vi "Read current vs temperature_3ch_2.1.vi"(8 "stop":bool) -> (0 "X3":cluster{"Y":dbl[], "Y":dbl[]}[](graph), 1 "Zx 4":cluster{"Y":dbl[], "Y":dbl[]}[](graph), 2 "Zx 3":cluster{"Y":dbl[], "Y":dbl[]}[](graph), 3 "Temp vs Time":cluster{"Y":dbl[], "Y":dbl[]}[](graph), 4 "i X":cluster{"Y":dbl[], "Y":dbl[]}[](graph), 5 "X 2":cluster{"Y":dbl[], "Y":dbl[]}[](graph))   [LabVIEW 2011]
uses:
  SubVI/ITX_Global.vi
  DAQ-lockin-SubVI/Source/Lock-in Globles.vi
panel:
  in  "Tab Control":T1(tab)
  in  "Lock-in # 2":u16(ring)=1 items=["Lock-in #1", "Lock-in #2", "Lock-in #3", "Lock-in #4"]
  out "OSC Configuration":T2(array[cluster])=[{"Signal Type"=enum."Sine Wave", "DC"=0.0005, "Amplitude"=0.001, "frequency"=1.346, "Phase"=0.0}, {"Signal Type"=enum."Sine Wave", "DC"=0.0, "Amplitude"=0.0, "frequency"=1.346, "Phase"=0.0}, {"Signal Type"=enum."Sine Wave", "DC"=0.0, "Amplitude"=0.0, "frequency"=1.346, "Phase"=0.0}, {"Signal Type"=enum."Sine Wave", "DC"=0.0, "Amplitude"=0.0, "frequency"=1.346, "Phase"=0.0}] {"frequency" format="%0.2p"; "Amplitude" format="%0.2p"; "DC" format="%.2p"}
  in  "Lock-in # 1":u16(ring) items=["Lock-in #1", "Lock-in #2", "Lock-in #3", "Lock-in #4"]
  in  "Lock-in # 3":u16(ring)=2 items=["Lock-in #1", "Lock-in #2", "Lock-in #3", "Lock-in #4"]
  in  "Lock-in # 4":u16(ring)=3 items=["Lock-in #1", "Lock-in #2", "Lock-in #3", "Lock-in #4"]
  in  "milliseconds to wait":u32=1000
  in  "Comments":string="SA02610M 20130128\ncool down\n"
  out "Connected":string="I-:4\nV2+:28\nI+:1\nV1+:2\nV-:3\nV2-:5\n"
  out "i Y":cluster{"Y":dbl[], "Y":dbl[]}[](graph)
  out "i X 3":cluster{"Y":dbl[], "Y":dbl[]}[](graph)
  out "i Y 3":cluster{"Y":dbl[], "Y":dbl[]}[](graph)
  out "Y 2":cluster{"Y":dbl[], "Y":dbl[]}[](graph)
  out "Y3":cluster{"Y":dbl[], "Y":dbl[]}[](graph)
  out "Zy 3":cluster{"Y":dbl[], "Y":dbl[]}[](graph)
  out "Zy 4":cluster{"Y":dbl[], "Y":dbl[]}[](graph)
  out "i X 2":cluster{"Y":dbl[], "Y":dbl[]}[](graph)
  out "i X 4":cluster{"Y":dbl[], "Y":dbl[]}[](graph)
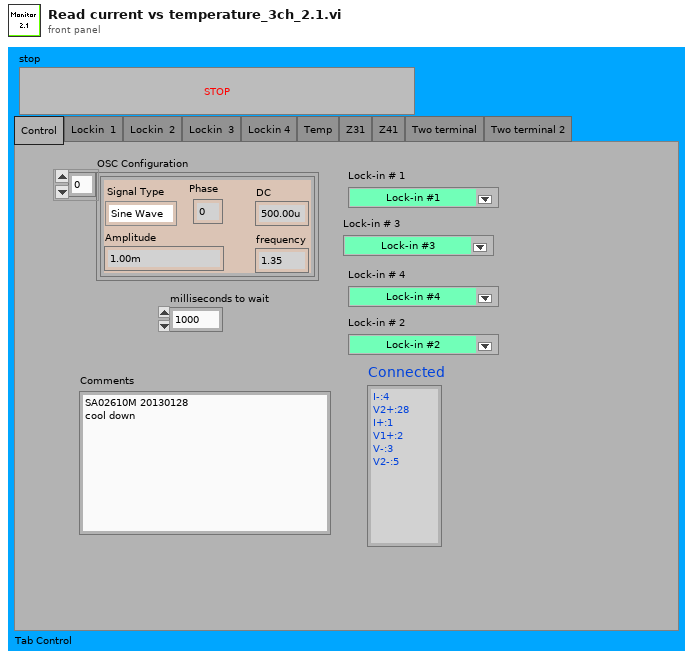
[diagram p1: front panel]
types:
  T1 = enum32{"Control", "Lockin  1", "Lockin  2", "Lockin  3", "Lockin 4", "Temp", "Z31", "Z41", "Two terminal", "Two terminal 2"}
  T2 = cluster{"Signal Type":enum16{"Sine Wave", "Triangle Wave", "Square Wave", "Sawtooth Wave"}, "DC":dbl, "Amplitude":dbl, "frequency":dbl, "Phase":dbl}[]
  T3 = cluster{"Signal Type":enum16{"Sine Wave", "Triangle Wave", "Square Wave", "Sawtooth Wave"}, "DC":dbl, "Amplitude":dbl, "frequency":dbl, "Phase":dbl}
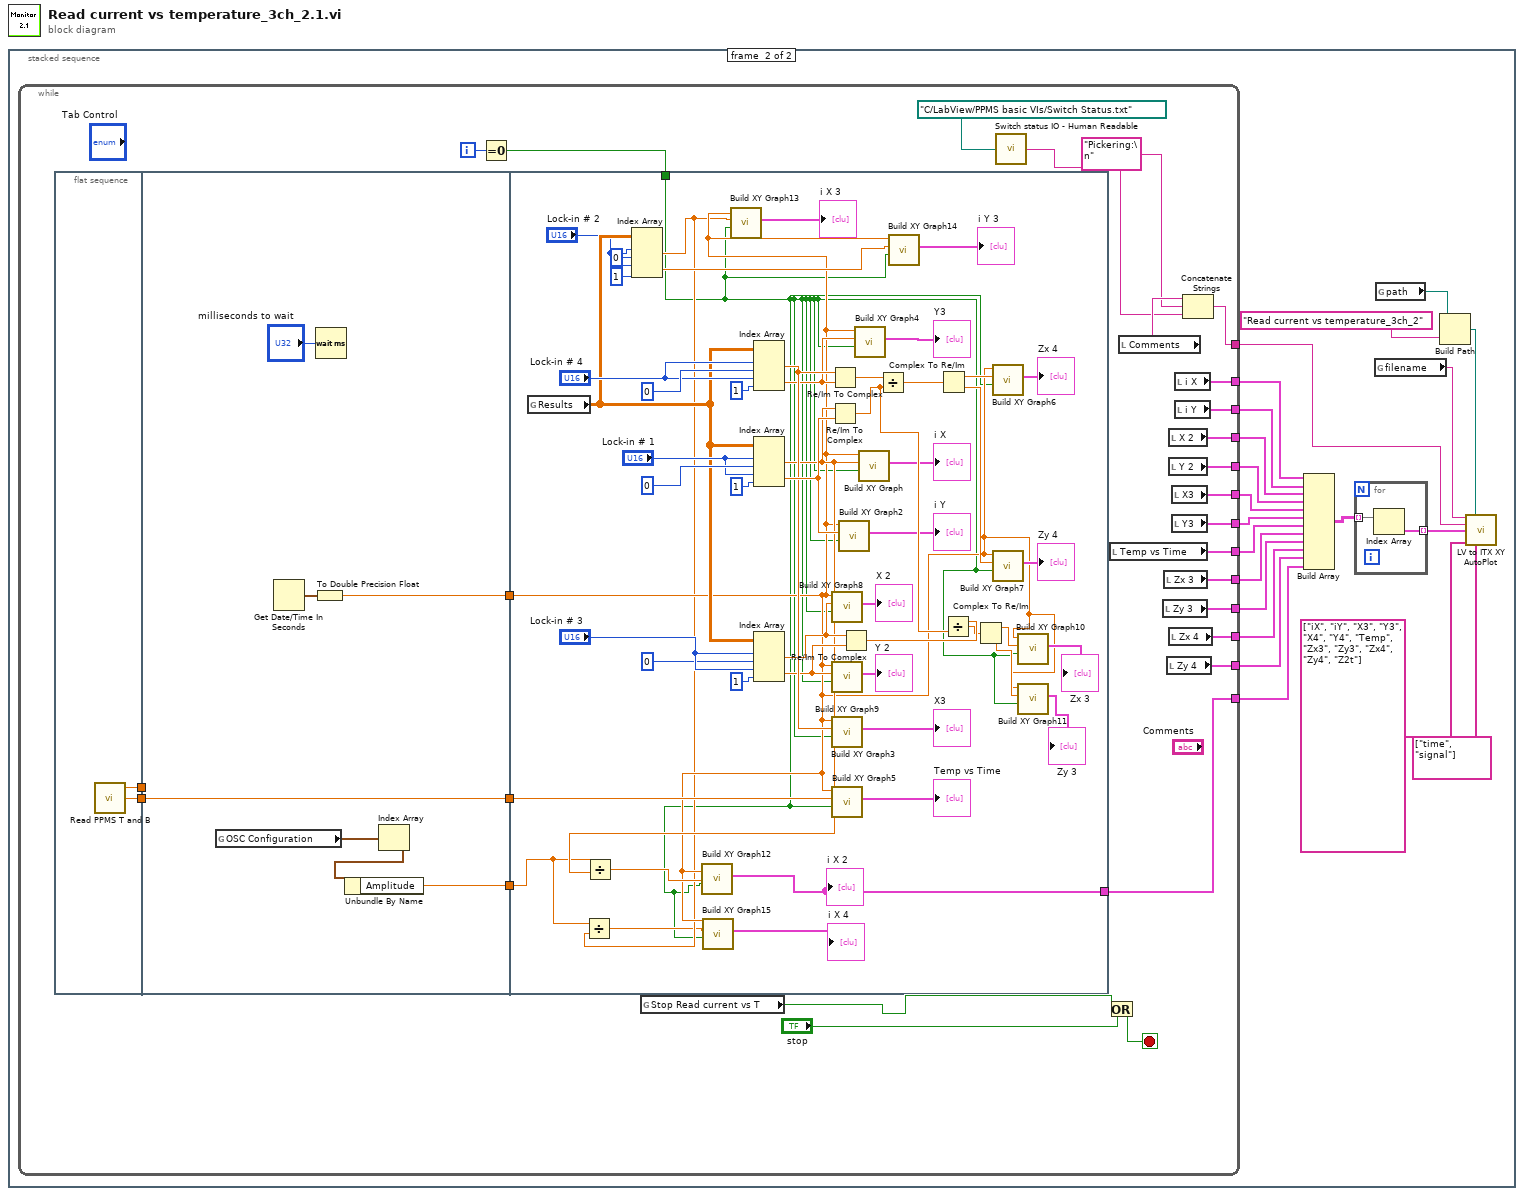
[diagram p0: block diagram]
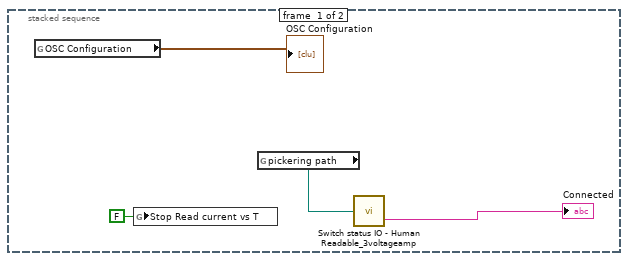
[diagram p2: hidden frame]
diagram:
  n1 = stacked-sequence {
    frame #0 {
      n2 = global read "Lock-in Globles.vi" "OSC Configuration"() -> (→"OSC Configuration":T2)
      n3 = global write "Lock-in Globles.vi" "Stop Read current vs T"(FALSE ("Stop Read current vs T")) -> ()
      n4 = global read "ITX_Global.vi" "pickering path"() -> (w1:path)
      n5 = call <userlib>:"Switch status IO - Human Readable_3voltageamp.vi"("Switch status"=w1) -> ("String"=→"Connected":string)  [unwired: 3 in]
    }
    frame #1 {
      n6 = while {
        tunnel: [w46] -> w25
        tunnel: [w45] -> w24
        tunnel: [w44] -> w23
        tunnel: [w43] -> w22
        tunnel: [w42] -> w21
        tunnel: [w41] -> w20
        tunnel: [w40] -> w19
        tunnel: [w39] -> w18
        tunnel: [w38] -> w17
        tunnel: [w37] -> w16
        tunnel: [w36] -> w15
        tunnel: [w34] -> w11
        tunnel: [w28] -> w5
        i -> [w52]
        stop <- w48 stop-if-true
        n7 = flat-sequence {
          tunnel: [w56] -> w53
          tunnel: [w55] -> w49
          tunnel: [w62] -> w54
          tunnel: w53 -> [w62]
          tunnel: [w60] -> w50
          tunnel: w49 -> [_]
          tunnel: [w57] -> w29
          tunnel: w54 -> [w96]
          tunnel: w51 -> [w65]
          tunnel: w50 -> [w69]
          tunnel: w29 -> [w68]
          tunnel: [w77] -> w28
          frame #0 {
            n8 = call "Read PPMS T and B.vi"() -> ("Temperature"=w56:dbl, "Time"=w55:dbl)  [unwired: 3 in, 1 out]
          }
          frame #1 {
            n9 = global read "Lock-in Globles.vi" "OSC Configuration"() -> (w59:T2)
            n10 = Get Date/Time In Seconds() -> (seconds since 1Jan1904=w61:timestamp)
            n11 = To Double Precision Float(number=w61) -> (double precision float=w60:dbl)
            n12 = Wait (ms)(milliseconds to wait="milliseconds to wait") -> ()  [unwired: 1 out]
            n13 = Index Array(array=w59) -> (element=w58:T3)  [unwired: 1 in]
            n14 = Unbundle By Name(w58) -> ("Amplitude"=w57:dbl)
          }
          frame #2 {
            n15 = global read "Lock-in Globles.vi" "Results"() -> (w76:dbl[][])
            n16 = Index Array(array=w76, index (row) #1="Lock-in # 2", index (col) #1=0 ("disabled index (col)"), index (row) #2="Lock-in # 2", index (col) #2=1 ("disabled index (col)")) -> (element #1=w67:dbl, element #2=w70:dbl)
            n17 = Divide(x=w68, y=w67) -> (x/y=w66:dbl)
            n18 = call "Build XY Graph15"("Reset"=w65, "Y Input"=w66, "X Input"=w69) -> ("XY Graph"=→"i X 4":cluster{"Y":dbl[], "Y":dbl[]}[])  [unwired: 2 in, 6 out]
            n19 = call "Build XY Graph13"("Reset"=w65, "Y Input"=w67, "X Input"=w69) -> ("XY Graph"=→"i X 3":cluster{"Y":dbl[], "Y":dbl[]}[])  [unwired: 2 in, 6 out]
            n20 = Index Array(array=w76, index (row) #1="Lock-in # 4", index (col) #1=0 ("disabled index (col)"), index (row) #2="Lock-in # 4", index (col) #2=1 ("disabled index (col)")) -> (element #1=w104:dbl, element #2=w103:dbl)
            n21 = Index Array(array=w76, index (row) #1="Lock-in # 1", index (col) #1=0 ("disabled index (col)"), index (row) #2="Lock-in # 1", index (col) #2=1 ("disabled index (col)")) -> (element #1=w79:dbl, element #2=w105:dbl)
            n22 = Divide(x=w68, y=w79) -> (x/y=w78:dbl)
            n23 = call "Build XY Graph12"("Reset"=w65, "Y Input"=w78, "X Input"=w69) -> ("XY Graph"=w77:cluster{"Y":dbl[], "Y":dbl[]}[])  [unwired: 2 in, 6 out]
            "i X 2" <- w77
            n24 = Index Array(array=w76, index (row) #1="Lock-in # 3", index (col) #1=0 ("disabled index (col)"), index (row) #2="Lock-in # 3", index (col) #2=1 ("disabled index (col)")) -> (element #1=w90:dbl, element #2=w89:dbl)
            n25 = Re/Im To Complex(1:w103, 2:w104) -> (0:w102:cdb)
            n26 = Re/Im To Complex(1:w105, 2:w79) -> (0:w87:cdb)
            n27 = call "Build XY Graph8"("Reset"=w65, "Y Input"=w90, "X Input"=w69) -> ("XY Graph"=→"X 2":cluster{"Y":dbl[], "Y":dbl[]}[])  [unwired: 2 in, 6 out]
            n28 = call "Build XY Graph9"("Reset"=w65, "Y Input"=w89, "X Input"=w69) -> ("XY Graph"=→"Y 2":cluster{"Y":dbl[], "Y":dbl[]}[])  [unwired: 2 in, 6 out]
            n29 = call "Build XY Graph3"("Reset"=w65, "Y Input"=w104, "X Input"=w69) -> ("XY Graph"=→"X3":cluster{"Y":dbl[], "Y":dbl[]}[])  [unwired: 2 in, 6 out]
            n30 = call "Build XY Graph5"("Reset"=w65, "Y Input"=w96, "X Input"=w69) -> ("XY Graph"=→"Temp vs Time":cluster{"Y":dbl[], "Y":dbl[]}[])  [unwired: 2 in, 6 out]
            n31 = call "Build XY Graph2"("Reset"=w65, "Y Input"=w105, "X Input"=w69) -> ("XY Graph"=→"i Y":cluster{"Y":dbl[], "Y":dbl[]}[])  [unwired: 2 in, 6 out]
            n32 = Re/Im To Complex(1:w89, 2:w90) -> (0:w88:cdb)
            n33 = call "Build XY Graph4"("Reset"=w65, "Y Input"=w103, "X Input"=w69) -> ("XY Graph"=→"Y3":cluster{"Y":dbl[], "Y":dbl[]}[])  [unwired: 2 in, 6 out]
            n34 = call "Build XY Graph"("Reset"=w65, "Y Input"=w79, "X Input"=w69) -> ("XY Graph"=→"i X":cluster{"Y":dbl[], "Y":dbl[]}[])  [unwired: 2 in, 6 out]
            n35 = Divide(x=w102, y=w87) -> (x/y=w101:cdb)
            n36 = call "Build XY Graph14"("Reset"=w65, "Y Input"=w70, "X Input"=w69) -> ("XY Graph"=→"i Y 3":cluster{"Y":dbl[], "Y":dbl[]}[])  [unwired: 2 in, 6 out]
            n37 = Complex To Re/Im(x + iy=w101) -> (x=w99:dbl, y=w100:dbl)
            n38 = Divide(x=w88, y=w87) -> (x/y=w86:cdb)
            n39 = Complex To Re/Im(x + iy=w86) -> (x=w85:dbl, y=w84:dbl)
            n40 = call "Build XY Graph6"("Reset"=w65, "Y Input"=w99, "X Input"=w69) -> ("XY Graph"=→"Zx 4":cluster{"Y":dbl[], "Y":dbl[]}[])  [unwired: 2 in, 6 out]
            n41 = call "Build XY Graph7"("Reset"=w65, "Y Input"=w100, "X Input"=w69) -> ("XY Graph"=→"Zy 4":cluster{"Y":dbl[], "Y":dbl[]}[])  [unwired: 2 in, 6 out]
            n42 = call "Build XY Graph10"("Reset"=w65, "Y Input"=w85, "X Input"=w69) -> ("XY Graph"=→"Zx 3":cluster{"Y":dbl[], "Y":dbl[]}[])  [unwired: 2 in, 6 out]
            n43 = call "Build XY Graph11"("Reset"=w65, "Y Input"=w84, "X Input"=w69) -> ("XY Graph"=→"Zy 3":cluster{"Y":dbl[], "Y":dbl[]}[])  [unwired: 2 in, 6 out]
          }
        }
        n44 = Equal To 0?(x=w52) -> (x = 0?=w51:bool)
        n45 = global read "Lock-in Globles.vi" "Stop Read current vs T"() -> (w30:bool)
        n46 = call <userlib>:"Switch status IO - Human Readable.vi"("Switch status"=path "C:/LabView/PPMS basic VIs/Switch Status.txt") -> ("String"=w31:string)
        n47 = Or(x=w30, y="stop") -> (x .or. y?=w48:bool)
        n48 = local read "Temp vs Time"() -> (w40:cluster{"Y":dbl[], "Y":dbl[]}[])
        n49 = local read "Comments"() -> (w33:string)
        n50 = local read "Zy 3"() -> (w38:cluster{"Y":dbl[], "Y":dbl[]}[])
        n51 = local read "Zx 3"() -> (w39:cluster{"Y":dbl[], "Y":dbl[]}[])
        n52 = local read "Zy 4"() -> (w36:cluster{"Y":dbl[], "Y":dbl[]}[])
        n53 = local read "X 2"() -> (w44:cluster{"Y":dbl[], "Y":dbl[]}[])
        n54 = local read "Y 2"() -> (w43:cluster{"Y":dbl[], "Y":dbl[]}[])
        n55 = local read "Zx 4"() -> (w37:cluster{"Y":dbl[], "Y":dbl[]}[])
        n56 = local read "X3"() -> (w42:cluster{"Y":dbl[], "Y":dbl[]}[])
        n57 = local read "Y3"() -> (w41:cluster{"Y":dbl[], "Y":dbl[]}[])
        n58 = local read "i X"() -> (w46:cluster{"Y":dbl[], "Y":dbl[]}[])
        n59 = local read "i Y"() -> (w45:cluster{"Y":dbl[], "Y":dbl[]}[])
        n60 = Concatenate Strings(w33, "Pickering:\n" ("string"), w31) -> (w34:string)
      }
      n61 = Build Array(w25, w24, w23, w22, w21, w20, w19, w18, w17, w16, w15, w5) -> (w14:cluster{"Y":dbl[], "Y":dbl[]}[][])
      n62 = for {
        tunnel: w14 -> [w27] mode=indexing
        tunnel: [w26] -> w13 mode=indexing
        n63 = Index Array(array=w27) -> (element=w26:cluster{"Y":dbl[], "Y":dbl[]})  [unwired: 1 in]
      }
      n64 = global read "ITX_Global.vi" "filename"() -> (w12:string)
      n65 = global read "ITX_Global.vi" "path"() -> (w8:path)
      n66 = Build Path(base path=w8, name or relative path="Read current vs temperature_3ch_2") -> (appended path=w7:path)
      n67 = call <userlib>:"LV to ITX XY AutoPlot.vi"("filename"=w12, "path"=w7, "Notes"=w11, "XY Array"=w13, "wavenames (.Vx, etc)"=string[] ["iX", "iY", "X3", "Y3", "X4", "Y4", "Temp", "Zx3", "Zy3", "Zx4", "Zy4", "Z2t"], "X,Y Labels"=string[] ["time", "signal"]) -> ()  [unwired: 9 in, 1 out]
    }
  }
